vi "test--Yellow.vi"(11 "Test Case In":refnum<class "Color to HSL.lvclass">) -> (0 "error out":errorcluster, 3 "Test Case Out":refnum<class "Color to HSL.lvclass">)   [LabVIEW 2021, in "Color to HSL.lvclass"]
uses:
  Color to HSL.lvclass
  C:/Program Files/National Instruments/LabVIEW 2024/vi.lib/Astemes/LUnit/Test Case.lvclass
  <vilib>/Astemes/LUnit/Test Case.lvclass/Test Case.ctl
  21945745-6a43-4f25-9869-c7df3bc0736d.vi
  2ebf1357-c1f7-433d-b8f9-8e277467dc7a.vi
  152675fc-8999-4eab-83f6-433c13dc1ec0.vi
  <vilib>/Astemes/LUnit/Core/LUnit Test Case/Private/Append Pass Result.vi
  <vilib>/Astemes/LUnit/Core/LUnit Test Case/Private/Append Fail Result.vi
  21945745-6a43-4f25-9869-c7df3bc0736d.vi/9c5d11cd-9439-4240-a1ee-d9baace9c924.vi
  2ebf1357-c1f7-433d-b8f9-8e277467dc7a.vi/9c5d11cd-9439-4240-a1ee-d9baace9c924.vi
  152675fc-8999-4eab-83f6-433c13dc1ec0.vi/9c5d11cd-9439-4240-a1ee-d9baace9c924.vi
  <vilib>/Astemes/LUnit/Core/LUnit Test Case/Private/Run In UI.vi
  <vilib>/Utility/error.llb/Clear Errors.vi
  <vilib>/Utility/colorconv.llb/Color to RGB.vi
  src/Material SubVIs/Material SubVIs.lvlib
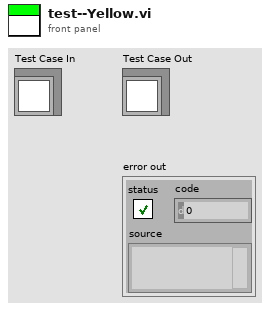
[diagram p1: front panel]
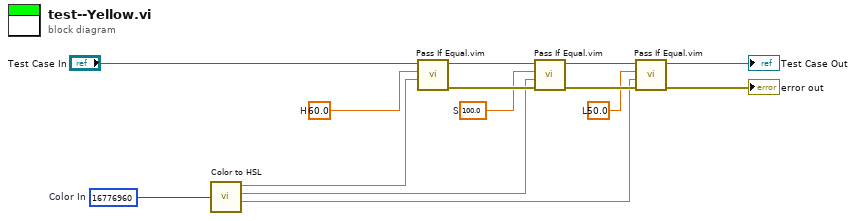
[diagram p0: block diagram]
diagram:
  w6 = 50.0  # L
  w7 = 100.0  # S
  w10 = 60.0  # H
  w11 = u32 16776960  # Color In
  n1 = call "Color to HSL.vi"("Color In"=w11) -> ("H (degrees)"=w4:dbl, "S (%)"=w3:dbl, "L (%)"=w2:dbl)  [unwired: 4 in, 1 out]
  n2 = call "Pass If Equal.vim"("Actual"=w4, "Expected"=w10, "LUnit Test Case In"="Test Case In") -> ("error out"=w13:errorcluster, "LUnit Test Case Out"=w9:refnum<class "Color to HSL.lvclass">)  [unwired: 7 in]
  n3 = call "Pass If Equal.vim"("error in (no error)"=w13, "Actual"=w3, "Expected"=w7, "LUnit Test Case In"=w9) -> ("error out"=w14:errorcluster, "LUnit Test Case Out"=w8:refnum<class "Color to HSL.lvclass">)  [unwired: 6 in]
  n4 = call "Pass If Equal.vim"("error in (no error)"=w14, "Actual"=w2, "Expected"=w6, "LUnit Test Case In"=w8) -> ("error out"=→"error out":errorcluster, "LUnit Test Case Out"=→"Test Case Out":refnum<class "Color to HSL.lvclass">)  [unwired: 6 in]
